vi "query NR HO UL_DL Center Channel Numebr.vi"(8 "error in (no error)":errorcluster caption="에러 입력(에러 없음)", 9 "Direction":T2, 10 "Selected CC Argements":T1, 11 "Anritsu Call Box 입력":refnum<class "Anritsu Call Box.lvclass">) -> (0 "error out":errorcluster caption="에러 출력", 2 "Center Channel Number":u32, 3 "Anritsu Call Box 출력":refnum<class "Anritsu Call Box.lvclass">)   [LabVIEW 2023, in "ANRITSU Call Box.lvlib" / "Anritsu Call Box.lvclass"]
uses:
  Anritsu Call Box.lvclass
  Type Definition/Uplink Downlink Enum.ctl
  ANRITSU Call Box.lvlib
  Type Definition/NR Selected CC Type Arguments.ctl
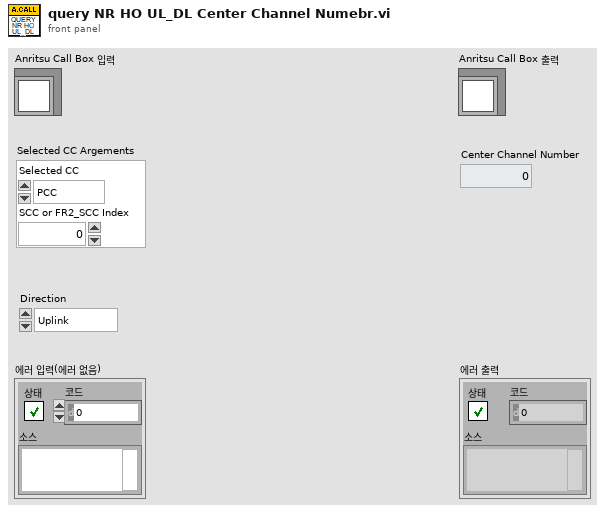
[diagram p1: front panel]
types:
  T1 = typedef "ANRITSU Call Box.lvlib/NR Selected CC Type Arguments.ctl" = cluster{"Selected CC":enum16{"PCC", "SCC", "FR2_PCC", "FR2_SCC"}, "SCC or FR2_SCC Index":u32}
  T2 = typedef "ANRITSU Call Box.lvlib/Uplink Downlink Enum.ctl" = enum16{"Uplink", "Downlink"}
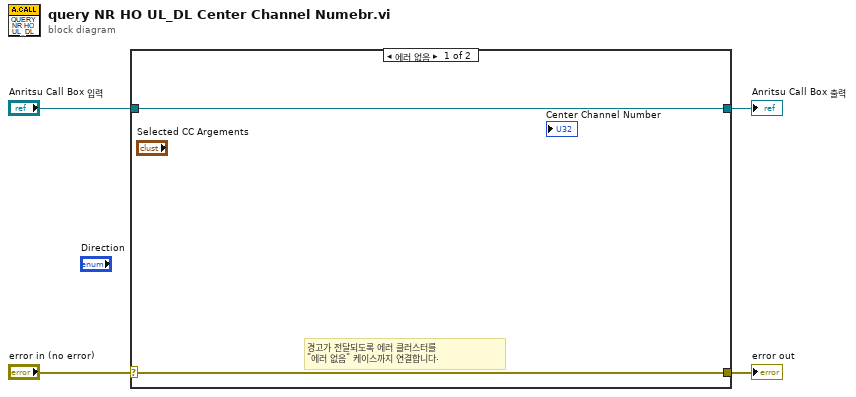
[diagram p0: block diagram]
diagram:
  n1 = case shown="에러 없음" "error in (no error)" {
    selector: "error in (no error)" -> [w5 w8]
    tunnel: [w5 w8] -> w3
    tunnel: [w6 w7] -> w1
    tunnel: "Anritsu Call Box 입력" -> [w6 w7]
    frame No Error {
      # "경고가 전달되도록 에러 클러스터를\n\"에러 없음\" 케이스까지 연결합니다."
    }
    frame Error {
    }
  }
  "error out" <- w3
  "Anritsu Call Box 출력" <- w1
